vi "Get Keys from Session .vi"(10 "Session Name":string, 11 "Device Settings":T1[](array[typedef])) -> (3 "Cluster":T2)   [LabVIEW 2021]
uses:
  TypeDefs/Device Settings.ctl
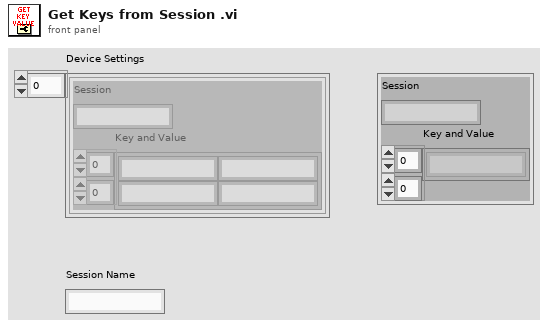
[diagram p1: front panel]
types:
  T1 = typedef "Device Settings.ctl" = cluster{"Session":string, "Key and Value":string[][]}
  T2 = cluster{"Session":string, "Key and Value":string[][]}
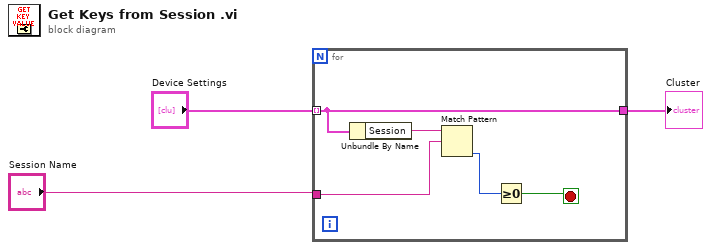
[diagram p0: block diagram]
diagram:
  n1 = for {
    tunnel: "Device Settings" -> [w4] mode=indexing
    tunnel: "Session Name" -> [w7]
    tunnel: [w4] -> w3
    stop <- w5 stop-if-true
    n2 = Unbundle By Name(w4) -> ("Session"=w8:string)
    n3 = Match Pattern(string=w8, regular expression=w7) -> (offset past match=w6:i32)  [unwired: 1 in, 3 out]
    n4 = Greater Or Equal To 0?(x=w6) -> (x >= 0?=w5:bool)
  }
  "Cluster" <- w3
